vi "Ajout_edition_segment EPC3000.vi"(5 "Action":enum16{"Edition", "Insertion", "Ajout"}(ring)=enum."Ajout", 7 "Numéro du segment":u8, 8 "Programme_entrée":cluster{"chaîne":string, "Valeur":dbl}[][](array[cluster]) {"Valeur" format="%#.1f"}, 9 "Valeur 2":dbl format="%#.1f", 10 "Valeur 1":dbl format="%#.1f", 11 "Type de segment/Valeur 0":u8) -> (0 "Programme_sortie":cluster{"chaîne":string, "Valeur":dbl}[][](array[cluster]) {"Valeur" format="%#.1f"})   [LabVIEW 2022 SP3]
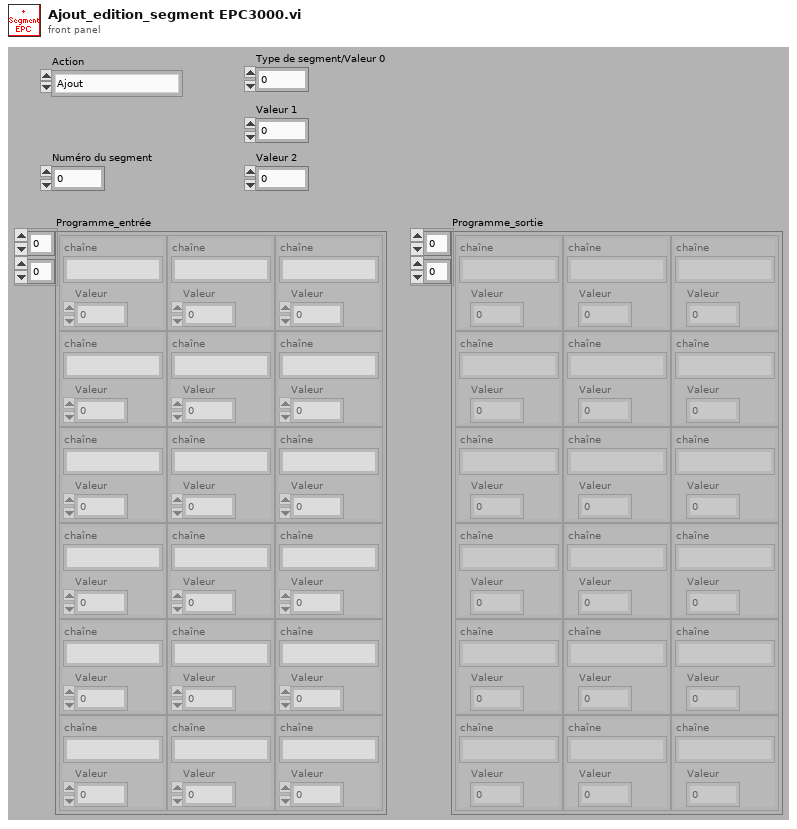
[diagram p1: front panel]
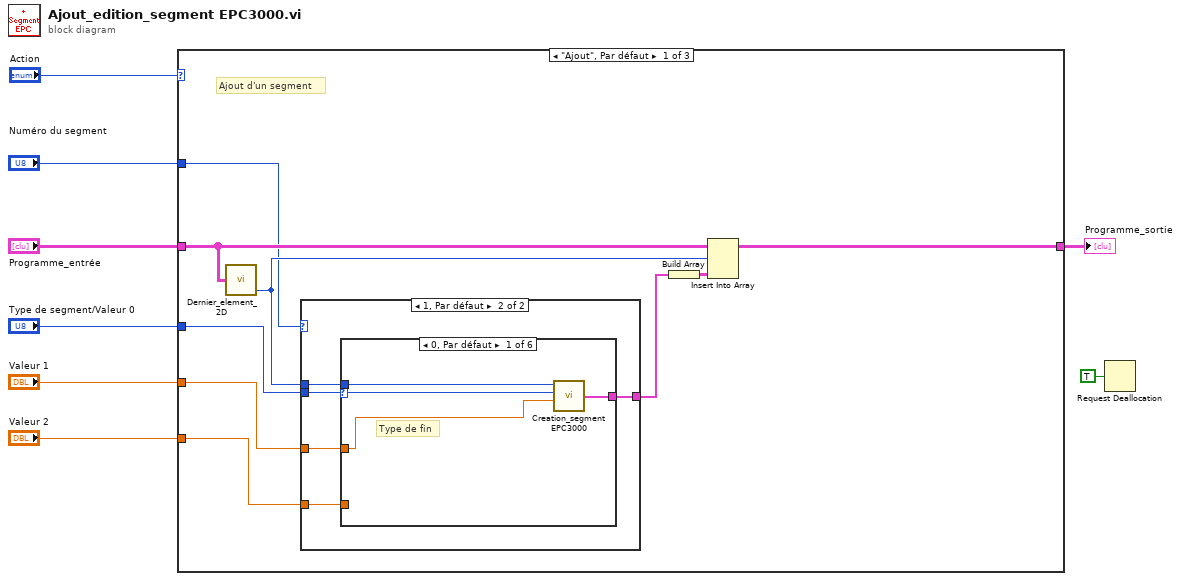
[diagram p0: block diagram]
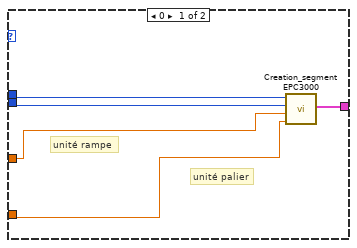
[diagram p2: hidden frame]
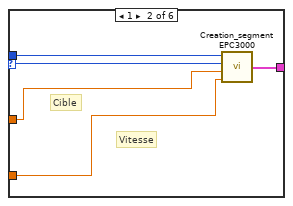
[diagram p3: hidden frame]
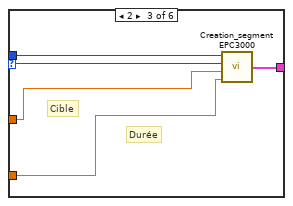
[diagram p4: hidden frame]
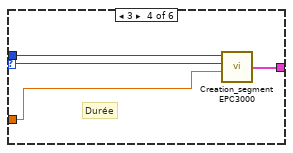
[diagram p5: hidden frame]
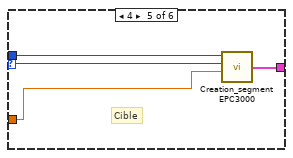
[diagram p6: hidden frame]
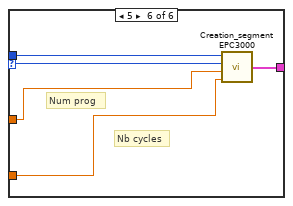
[diagram p7: hidden frame]
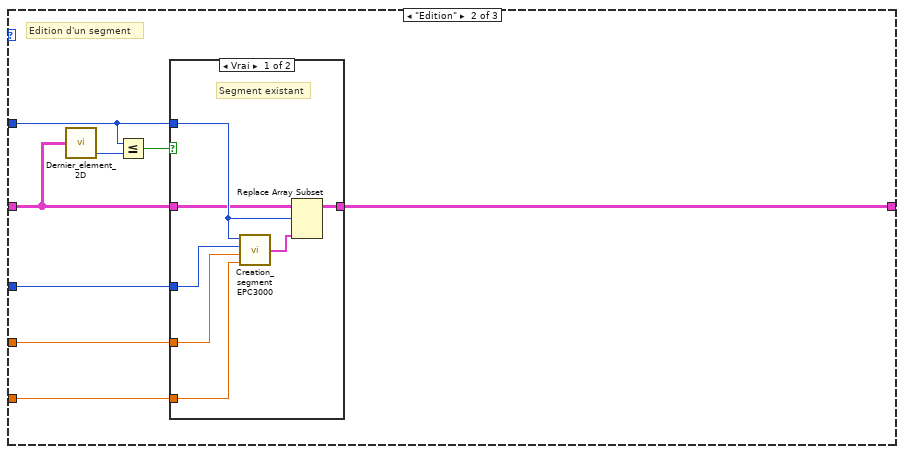
[diagram p8: hidden frame]
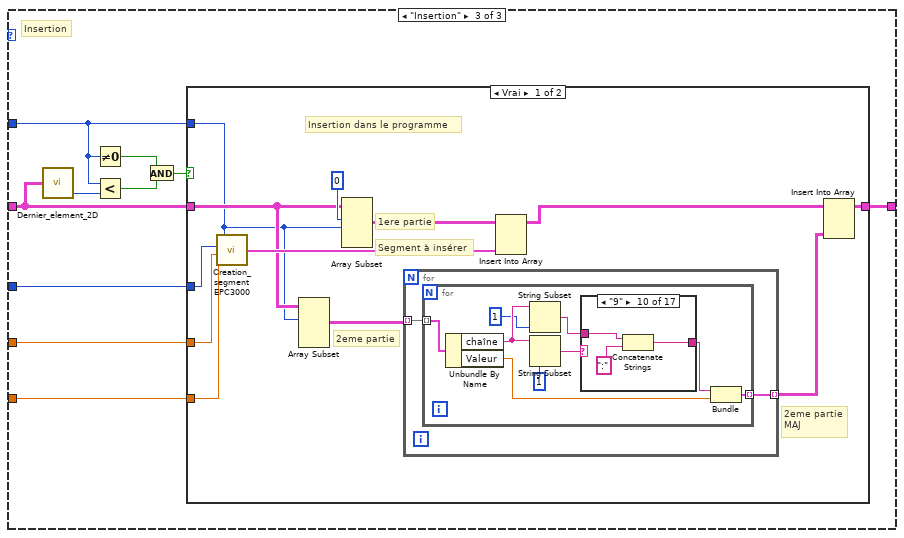
[diagram p10: hidden frame]
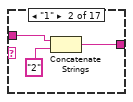
[diagram p12: hidden frame]
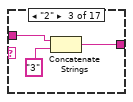
[diagram p13: hidden frame]
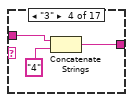
[diagram p14: hidden frame]
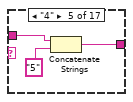
[diagram p15: hidden frame]
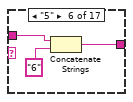
[diagram p16: hidden frame]
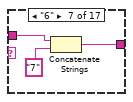
[diagram p17: hidden frame]
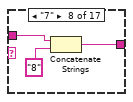
[diagram p18: hidden frame]
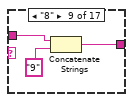
[diagram p19: hidden frame]
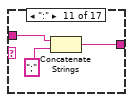
[diagram p20: hidden frame]
diagram:
  n1 = case shown="\"Ajout\", Par défaut" "Action" {
    tunnel: "Programme_entrée" -> [w11 w59 w75]
    tunnel: [w15 w55 w80] -> w3
    tunnel: "Numéro du segment" -> [w9 w60 w74]
    tunnel: "Type de segment/Valeur 0" -> [w14 w58 w79]
    tunnel: "Valeur 1" -> [w13 w57 w78]
    tunnel: "Valeur 2" -> [w12 w56 w77]
    frame "Ajout", Default {
      # "Ajout d'un segment"
      n2 = call "Dernier_element_2D.vi"("Programme"=w11) -> ("Taille/Indice N+1"=w10:i32)  [unwired: 2 out]
      n3 = case shown="1, Par défaut" w9 {
        tunnel: [w22 w27] -> w16
        tunnel: w14 -> [w20 w26]
        tunnel: w13 -> [w19 w25]
        tunnel: w12 -> [w18 w24]
        tunnel: w10 -> [w21 w23]
        frame 0 {
          # "unité palier"
          # "unité rampe"
          n4 = call "Creation_segment EPC3000.vi"("Valeur 2"=w18, "Valeur 1"=w19, "Type de segment/Valeur 0"=w20, "Numéro de segment"=w21) -> ("Segment"=w22:cluster{"chaîne p":string, "Valeur 1":dbl}[])
        }
        frame 1, Default {
          n5 = case shown="0, Par défaut" w26 {
            selector: w26 -> [w30 w35 w40 w44 w48 w53]
            tunnel: w23 -> [w31 w36 w41 w45 w49 w54]
            tunnel: [w29 w34 w39 w43 w47 w52] -> w27
            tunnel: w25 -> [w28 w33 w38 w42 w46 w51]
            tunnel: w24 -> [_ w32 w37 _ _ w50]
            frame 0, Default {
              # "Type de fin"
              n6 = call "Creation_segment EPC3000.vi"("Valeur 1"=w28, "Type de segment/Valeur 0"=w30, "Numéro de segment"=w31) -> ("Segment"=w29:cluster{"chaîne p":string, "Valeur 1":dbl}[])  [unwired: 1 in]
            }
            frame 1 {
              # "Vitesse"
              # "Cible"
              n7 = call "Creation_segment EPC3000.vi"("Valeur 2"=w32, "Valeur 1"=w33, "Type de segment/Valeur 0"=w35, "Numéro de segment"=w36) -> ("Segment"=w34:cluster{"chaîne p":string, "Valeur 1":dbl}[])
            }
            frame 2 {
              # "Durée"
              # "Cible"
              n8 = call "Creation_segment EPC3000.vi"("Valeur 2"=w37, "Valeur 1"=w38, "Type de segment/Valeur 0"=w40, "Numéro de segment"=w41) -> ("Segment"=w39:cluster{"chaîne p":string, "Valeur 1":dbl}[])
            }
            frame 3 {
              # "Durée"
              n9 = call "Creation_segment EPC3000.vi"("Valeur 1"=w42, "Type de segment/Valeur 0"=w44, "Numéro de segment"=w45) -> ("Segment"=w43:cluster{"chaîne p":string, "Valeur 1":dbl}[])  [unwired: 1 in]
            }
            frame 4 {
              # "Cible"
              n10 = call "Creation_segment EPC3000.vi"("Valeur 1"=w46, "Type de segment/Valeur 0"=w48, "Numéro de segment"=w49) -> ("Segment"=w47:cluster{"chaîne p":string, "Valeur 1":dbl}[])  [unwired: 1 in]
            }
            frame 5 {
              # "Num prog"
              # "Nb cycles"
              n11 = call "Creation_segment EPC3000.vi"("Valeur 2"=w50, "Valeur 1"=w51, "Type de segment/Valeur 0"=w53, "Numéro de segment"=w54) -> ("Segment"=w52:cluster{"chaîne p":string, "Valeur 1":dbl}[])
            }
          }
        }
      }
      n12 = Build Array(w16) -> (w17:cluster{"chaîne p":string, "Valeur 1":dbl}[][])
      n13 = Insert Into Array(array=w11, index (row)=w10, new element=w17) -> (w15:cluster{"chaîne":string, "Valeur":dbl}[][])  [unwired: 1 in]
    }
    frame "Edition" {
      # "Edition d'un segment"
      n14 = call "Dernier_element_2D.vi"("Programme"=w59) -> ("Taille/Indice N+1"=w61:i32)  [unwired: 2 out]
      n15 = Less Or Equal?(x=w60, y=w61) -> (x <= y?=w62:bool)
      n16 = case shown="Vrai" w62 {
        tunnel: w59 -> [w63 w70]
        tunnel: [w68 w70] -> w55
        tunnel: w60 -> [w64 _]
        tunnel: w58 -> [w65 _]
        tunnel: w57 -> [w66 _]
        tunnel: w56 -> [w67 _]
        frame True {
          # "Segment existant"
          n17 = call "Creation_segment EPC3000.vi"("Valeur 2"=w67, "Valeur 1"=w66, "Type de segment/Valeur 0"=w65, "Numéro de segment"=w64) -> ("Segment"=w69:cluster{"chaîne p":string, "Valeur 1":dbl}[])
          n18 = Replace Array Subset(array=w63, new element=w69, index (row)=w64) -> (w68:cluster{"chaîne":string, "Valeur":dbl}[][])  [unwired: 1 in]
        }
        frame False {
          # "Segment inexistant"
        }
      }
    }
    frame "Insertion" {
      # "Insertion"
      n19 = call "Dernier_element_2D.vi"("Programme"=w75) -> ("Taille/Indice N+1"=w76:i32)  [unwired: 2 out]
      n20 = Not Equal To 0?(x=w74) -> (x != 0?=w72:bool)
      n21 = Less?(x=w74, y=w76) -> (x < y?=w73:bool)
      n22 = And(x=w72, y=w73) -> (x .and. y?=w71:bool)
      n23 = case shown="Vrai" w71 {
        tunnel: w75 -> [w84 w151]
        tunnel: [w85 w151] -> w80
        tunnel: w74 -> [w83 _]
        tunnel: w79 -> [w90 _]
        tunnel: w78 -> [w91 _]
        tunnel: w77 -> [w92 _]
        frame True {
          # "2eme partie\nMAJ"
          # "Segment à insérer"
          # "2eme partie"
          # "1ere partie"
          # "Insertion dans le programme"
          n24 = call "Creation_segment EPC3000.vi"("Valeur 2"=w92, "Valeur 1"=w91, "Type de segment/Valeur 0"=w90, "Numéro de segment"=w83) -> ("Segment"=w87:cluster{"chaîne p":string, "Valeur 1":dbl}[])
          n25 = Array Subset(array=w84, index (row)=w83) -> (w82:cluster{"chaîne":string, "Valeur":dbl}[][])  [unwired: 3 in]
          n26 = Array Subset(array=w84, index (row)=0 ("indice"), length (row)=w83) -> (w88:cluster{"chaîne":string, "Valeur":dbl}[][])  [unwired: 2 in]
          n27 = for {
            tunnel: w82 -> [w94] mode=indexing
            tunnel: [w93] -> w81 mode=indexing
            n28 = for {
              tunnel: w94 -> [w103] mode=indexing
              tunnel: [w95] -> w93 mode=indexing
              n29 = Unbundle By Name(w103) -> ("chaîne"=w99:string, "Valeur"=w100:dbl)
              n30 = String Subset(string=w99, length (rest)=1 ("longueur (reste)")) -> (substring=w97:string)  [unwired: 1 in]
              n31 = String Subset(string=w99, offset (0)=1) -> (substring=w101:string)  [unwired: 1 in]
              n32 = case shown="\"9\"" w101 {
                tunnel: w97 -> [w104 w106 w109 w112 w115 w118 w121 w124 w127 w130 w133 w136 w139 w142 w145 w148 w150]
                tunnel: [w104 w105 w108 w111 w114 w117 w120 w123 w126 w129 w132 w135 w138 w141 w144 w147 w150] -> w96
                frame Default {
                  # "n'arrive jamais"
                }
                frame "1" {
                  n33 = Concatenate Strings(w106, "2") -> (w105:string)
                }
                frame "2" {
                  n34 = Concatenate Strings(w109, "3") -> (w108:string)
                }
                frame "3" {
                  n35 = Concatenate Strings(w112, "4") -> (w111:string)
                }
                frame "4" {
                  n36 = Concatenate Strings(w115, "5") -> (w114:string)
                }
                frame "5" {
                  n37 = Concatenate Strings(w118, "6") -> (w117:string)
                }
                frame "6" {
                  n38 = Concatenate Strings(w121, "7") -> (w120:string)
                }
                frame "7" {
                  n39 = Concatenate Strings(w124, "8") -> (w123:string)
                }
                frame "8" {
                  n40 = Concatenate Strings(w127, "9") -> (w126:string)
                }
                frame "9" {
                  n41 = Concatenate Strings(w130, ":") -> (w129:string)
                }
                frame ":" {
                  n42 = Concatenate Strings(w133, ";") -> (w132:string)
                }
                frame ";" {
                  n43 = Concatenate Strings(w136, "<") -> (w135:string)
                }
                frame "<" {
                  n44 = Concatenate Strings(w139, "=") -> (w138:string)
                }
                frame "=" {
                  n45 = Concatenate Strings(w142, ">") -> (w141:string)
                }
                frame ">" {
                  n46 = Concatenate Strings(w145, "?") -> (w144:string)
                }
                frame "?" {
                  n47 = Concatenate Strings(w148, "@") -> (w147:string)
                }
                frame "@" {
                  # "n'arrive jamais"
                }
              }
              n48 = Bundle("chaîne"=w96, "Valeur"=w100) -> (w95:cluster{"chaîne":string, "Valeur":dbl})  [unwired: 1 in]
            }
          }
          n49 = Insert Into Array(array=w88, new element=w87) -> (w86:cluster{"chaîne":string, "Valeur":dbl}[][])  [unwired: 2 in]
          n50 = Insert Into Array(array=w86, new element=w81) -> (w85:cluster{"chaîne":string, "Valeur":dbl}[][])  [unwired: 2 in]
        }
        frame False {
          # "Inutile d'insérer en dehors du programme"
          # "On recopie le programme sans le modifier"
        }
      }
    }
  }
  "Programme_sortie" <- w3
  n51 = Request Deallocation(TRUE ("flag")) -> ()
